vi "Add Virtual Curve.vi"(8 "error in (no error)":errorcluster, 11 "Data Viewer in":refnum<class "Data Viewer.lvclass">) -> (0 "error out":errorcluster, 1 "Cancel?":bool, 3 "Data Viewer out":refnum<class "Data Viewer.lvclass">)   [LabVIEW 2020, in "Data Viewer.lvlib" / "Data Viewer.lvclass"]
uses:
  Data Viewer.lvclass
  Data Viewer.lvclass/Data Viewer.ctl
panel:
  in  "Tab Control":enum32{"Page 2"}(tab)
  in  "Add Virtual Curve":bool
  in  "曲线B":u16(ring) items=["1 sample", "2 sample", "3 ", "4 "]
  in  "曲线A":u16(ring) items=["1 sample", "2 sample", "3 ", "4 "]
  in  "操作":enum16{"A-B", "B-A", "A+B"}(ring)
  in  "目标曲线":u16(ring) items=["1", "2", "3", "4"]
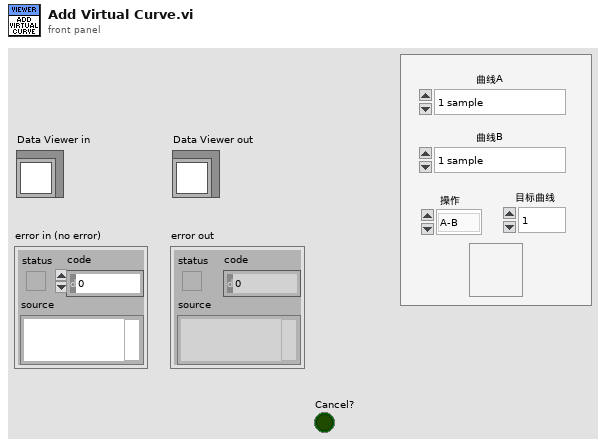
[diagram p1: front panel]
types:
  T1 = enum32{"Invalid", "Standard", "Closed", "Hidden", "Minimized", "Maximized"}
  T2 = typedef "Data Viewer.lvlib/Data Viewer.lvclass/Plot Property--cluster.ctl" = cluster{"Name":string, "Visible":bool, "Color":u32, "Scale Index":i32, "Show Peak Line":bool}
  T3 = typedef "Data Viewer.lvlib/Data Serie--cluster.ctl" = cluster{"Name":string, "Unit":string, "Sample Rate[Hz]":dbl, "Delta t[S]":dbl, "t0":timestamp, "Length":i32, "Time":timestamp[], "Value":dbl[]}
  T4 = cluster{"Name":string, "Scale":u16, "Color":u32, "Visible":bool, "Peak Line":bool}[]
  T5 = cluster{"Name":string, "Scale":u16, "Color":u32, "Visible":bool, "Peak Line":bool}
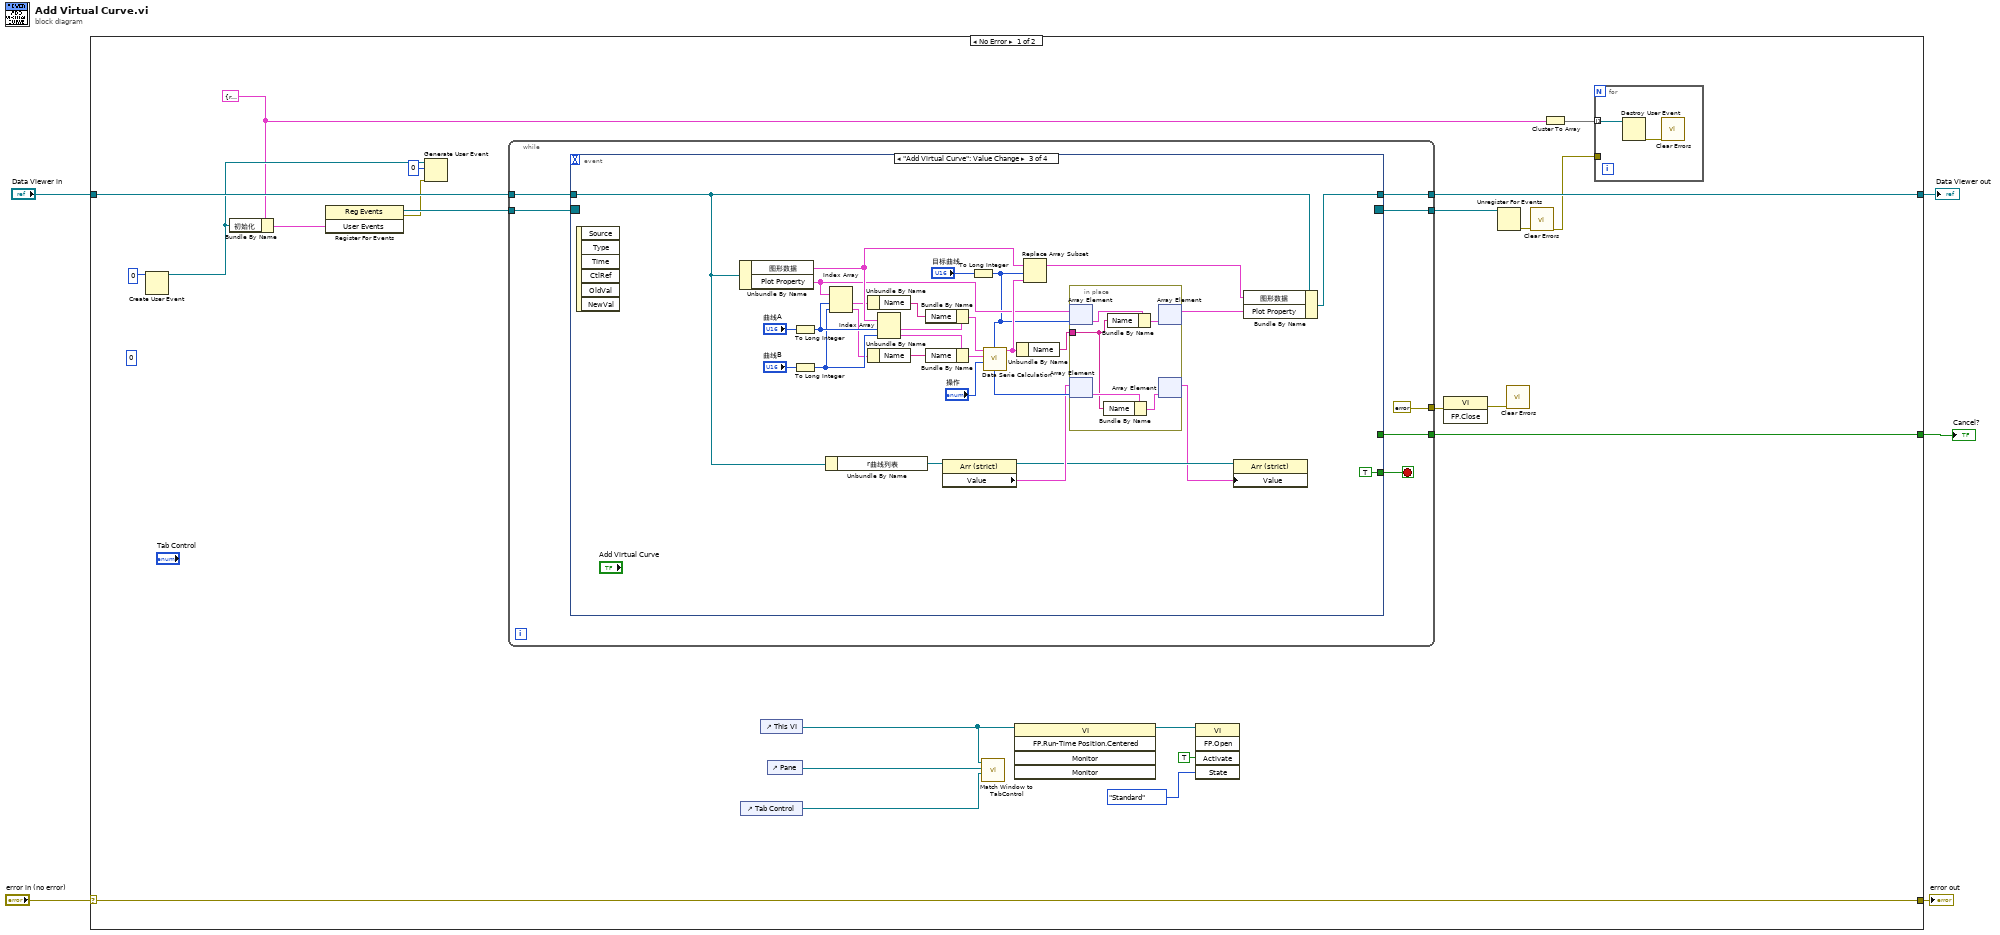
[diagram p0: block diagram]
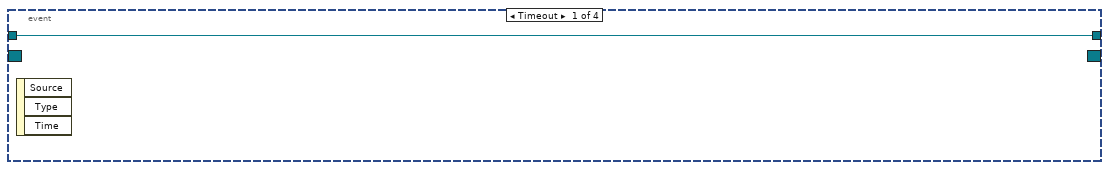
[diagram p2: hidden frame]
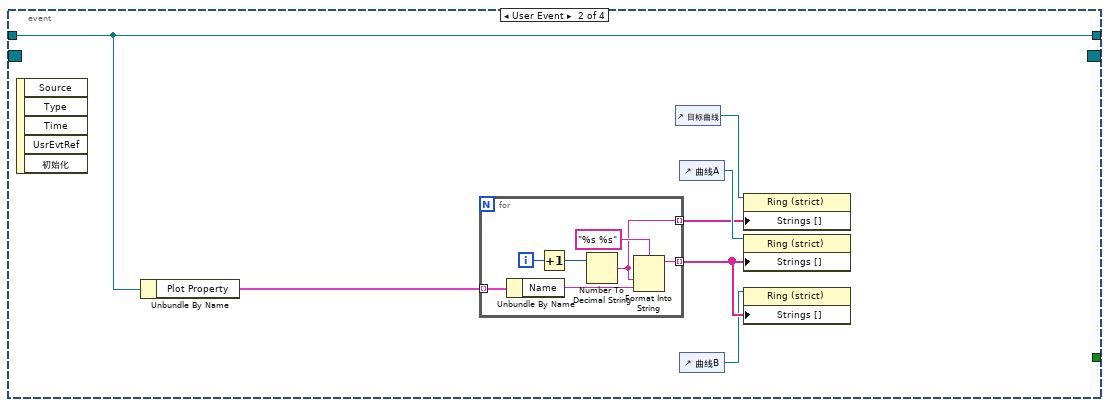
[diagram p3: hidden frame]
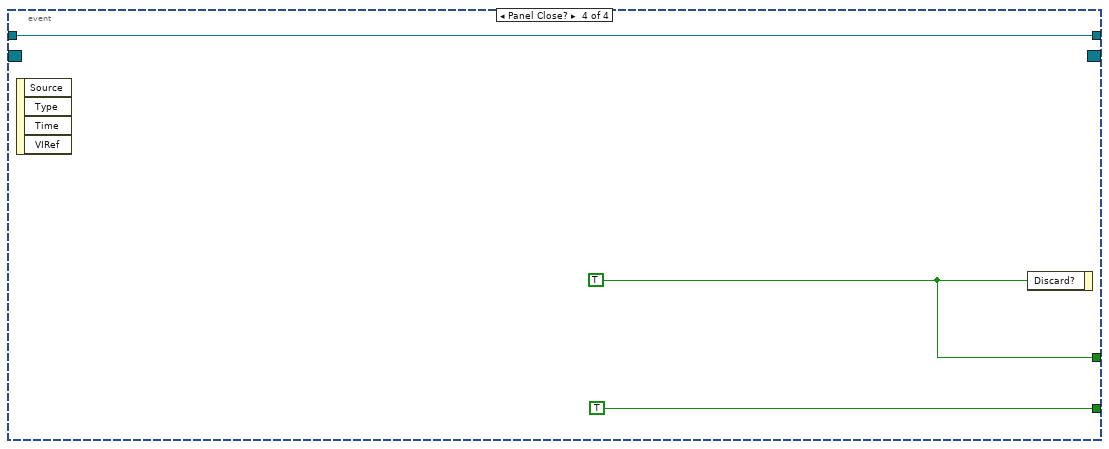
[diagram p4: hidden frame]
diagram:
  n1 = case shown="No Error" "error in (no error)" {
    selector: "error in (no error)" -> [w28 w90]
    tunnel: [w28 w90] -> w4
    tunnel: [w20 w89] -> w2
    tunnel: "Data Viewer in" -> [w21 w89]
    tunnel: [w17 _] -> w1
    frame No Error {
      w10 = cluster{"初始化":refnum<user-event>} {"初始化"=refnum} ("User Events")
      (unwired) 0
      n2 = Create User Event(user event datatype=0 ("初始化")) -> (user event=w13:refnum<user-event>)  [unwired: 1 in, 1 out]
      n3 = Bundle By Name(cluster=w10, "初始化"=w13) -> (w15:cluster{"初始化":refnum<user-event>})
      n4 = register-events(w15) -> (reference out=w14:refnum<event-registration>, error out=w12:errorcluster)  [unwired: 2 in]
      n5 = Generate User Event(user event=w13, event data cluster=0 ("event data"), error in=w12) -> ()  [unwired: 1 in, 2 out]
      n6 = while {
        tunnel: w21 -> [w36]
        tunnel: [w35] -> w20
        tunnel: [errorcluster {"status"=FALSE, "code"=0, "source"=""} ("error in (no error)")] -> w19
        tunnel: [w33] -> w17
        tunnel: w14 -> [w32]
        tunnel: [w31] -> w9
        stop <- w37 stop-if-true
        n7 = event shown="[2] \"Add Virtual Curve\": Value Change" {
          selector: w32 -> [_ _ _ _]
          dyn-events: [_ _ _ _] -> w31
          timeout: _ -> [_ _ _ _]
          tunnel: [_ _ TRUE TRUE] -> w37
          tunnel: [w38 w45 w77 w87] -> w35
          tunnel: w36 -> [w38 w45 w60 w87]
          tunnel: [_ _ _ w86] -> w33
          event Timeout {
            n8 = event-data() -> ()  [unwired: 1 in, 3 out]
          }
          event User Event {
            n9 = event-data() -> ()  [unwired: 1 in, 5 out]
            n10 = Unbundle By Name(w45) -> ("Plot Property"=w44:T2[])
            n11 = for {
              tunnel: w44 -> [w52] mode=indexing
              tunnel: [w48] -> w42 mode=indexing
              tunnel: [w46] -> w39 mode=indexing
              i -> [w51]
              n12 = Unbundle By Name(w52) -> ("Name"=w50:string)
              n13 = Increment(x=w51) -> (x+1=w47:i32)
              n14 = Number To Decimal String(number=w47) -> (decimal integer string=w46:string)  [unwired: 1 in]
              n15 = Format Into String(format string="%s %s", w46, w50) -> (resulting string=w48:string)  [unwired: 2 in, 1 out]
            }
            n16 = control-ref of="目标曲线"() -> (w40:refnum<vi>)
            n17 = control-ref of="曲线A"() -> (w43:refnum<vi>)
            n18 = control-ref of="曲线B"() -> (w41:refnum<vi>)
            n19 = property class="Ring (strict)"(reference=w40, "Strings []"=w39) -> ()  [unwired: 1 in, 2 out]
            n20 = property class="Ring (strict)"(reference=w43, "Strings []"=w42) -> ()  [unwired: 1 in, 2 out]
            n21 = property class="Ring (strict)"(reference=w41, "Strings []"=w42) -> ()  [unwired: 1 in, 2 out]
          }
          event "Add Virtual Curve": Value Change {
            n22 = event-data() -> ()  [unwired: 1 in, 6 out]
            n23 = Unbundle By Name(w60) -> ("图形数据"=w76:T3[], "Plot Property"=w70:T2[])
            n24 = To Long Integer(number="曲线A") -> (32bit integer=w69:i32)
            n25 = To Long Integer(number="曲线B") -> (32bit integer=w68:i32)
            n26 = Unbundle By Name(w60) -> ("r曲线列表"=w59:refnum<vi>)
            n27 = Index Array(array=w70, index #1=w69, index #2=w68) -> (element #1=w67:T2, element #2=w64:T2)
            n28 = Unbundle By Name(w67) -> ("Name"=w66:string)
            n29 = Unbundle By Name(w64) -> ("Name"=w65:string)
            n30 = Index Array(array=w76, index #1=w69, index #2=w68) -> (element #1=w71:T3, element #2=w63:T3)
            n31 = Bundle By Name(cluster=w71, "Name"=w66) -> (w62:T3)
            n32 = Bundle By Name(cluster=w63, "Name"=w65) -> (w61:T3)
            n33 = property class="Arr (strict)"(reference=w59) -> (reference out=w55:refnum<vi>, "Value"=w56:T4)  [unwired: 1 in, 1 out]
            n34 = To Long Integer(number="目标曲线") -> (32bit integer=w57:i32)
            n35 = call "Data Serie Calculation.vi"("Operation"="操作", "Data Serie B"=w61, "Data Serie A"=w62) -> ("Data Serie Out"=w73:T3)  [unwired: 7 in, 1 out]
            n36 = Unbundle By Name(w73) -> ("Name"=w58:string)
            n37 = Replace Array Subset(array=w76, new element=w73, index=w57) -> (w75:T3[])
            n38 = in-place {
              in-place-border: w58 -> [w82]
              n39 = in-place-array #1(w70, w57) -> (w85:T2)
              n40 = in-place-array #2(w56, w57) -> (w83:T5)
              n41 = Bundle By Name(cluster=w83, "Name"=w82) -> (w81:T5)
              n42 = Bundle By Name(cluster=w85, "Name"=w82) -> (w84:T2)
              n43 = in-place-array #1(w84) -> (w72:T2[])  [unwired: 1 out]
              n44 = in-place-array #2(w81) -> (w54:T4)  [unwired: 1 out]
            }
            n45 = property class="Arr (strict)"(reference=w55, "Value"=w54) -> ()  [unwired: 1 in, 2 out]
            n46 = Bundle By Name(cluster=w60, "图形数据"=w75, "Plot Property"=w72) -> (w77:refnum<class "Data Viewer.lvclass">)
          }
          event Panel Close? {
            w86 = TRUE ("Discard?")
            n47 = event-data() -> ()  [unwired: 1 in, 4 out]
            n48 = event-data("Discard?"=w86) -> ()  [unwired: 1 in, 1 out]
          }
        }
      }
      n49 = control-ref of="Tab Control"() -> (w27:refnum<vi>)
      n50 = control-ref of="This VI"() -> (w25:refnum<vi>)
      n51 = control-ref of="Pane"() -> (w26:refnum<vi>)
      n52 = call "Match Window to TabControl.vi"("Tab Control"=w27, "Pane"=w26, "VI in"=w25) -> ()  [unwired: 9 in]
      n53 = invoke class="VI" method="FP.Run-Time Position.Centered"(reference=w25) -> (reference out=w24:refnum<vi>)  [unwired: 4 in, 4 out]
      n54 = invoke class="VI" method="FP.Open"(reference=w24, "Activate"=TRUE ("Activate?"), "State"=T1."Standard") -> ()  [unwired: 2 in, 5 out]
      n55 = invoke class="VI" method="FP.Close"(error in=w19) -> (error out=w18:errorcluster)  [unwired: 2 in, 2 out]
      n56 = Unregister For Events(event registration refnum=w9) -> (error out=w8:errorcluster)  [unwired: 1 in]
      n57 = call <vilib>:"Clear Errors.vi"("error in (no error)"=w18) -> ()  [unwired: 5 in, 2 out]
      n58 = call <vilib>:"Clear Errors.vi"("error in (no error)"=w8) -> ("error out"=w6:errorcluster)  [unwired: 5 in, 1 out]
      n59 = Cluster To Array(cluster=w10) -> (array=w7:refnum<user-event>[])
      n60 = for {
        tunnel: w7 -> [w30] mode=indexing
        tunnel: w6 -> [_]
        n61 = Destroy User Event(user event=w30) -> (error out=w29:errorcluster)  [unwired: 1 in]
        n62 = call <vilib>:"Clear Errors.vi"("error in (no error)"=w29) -> ()  [unwired: 5 in, 2 out]
      }
    }
    frame Error {
    }
  }
  "error out" <- w4
  "Data Viewer out" <- w2
  "Cancel?" <- w1
